vi "Read Boolean Channel Properties.vi"(7 "Input?":bool, 8 "error in (no error)":errorcluster, 10 "Bool Channel ID":string, 11 "Channel in":refnum<class "Channel.lvclass">) -> (0 "error out":errorcluster, 2 "Boolean Channel":T1, 3 "Channel out":refnum<class "Channel.lvclass">)   [LabVIEW 2026, in "Modbus.lvlib" / "Modbus.lvclass"]
uses:
  Modbus.lvclass
  <vilib>/FlexLogger/SDK/PluginSDK.lvlibp/PEFClasses/SDK/Channel/Channel.lvclass
  Types/Boolean Data.ctl
  Types/Modbus Table.ctl
  Globals/Modbus Strings.vi
  <vilib>/FlexLogger/SDK/PluginSDK.lvlibp/PEFClasses/SDK/Channel/ParameterAccess/Read Enum.vi
  <vilib>/FlexLogger/SDK/PluginSDK.lvlibp/PEFClasses/SDK/Channel/ParameterAccess/Read I32.vi
  <vilib>/FlexLogger/SDK/PluginSDK.lvlibp/PEFClasses/SDK/Channel/Read Valid.vi
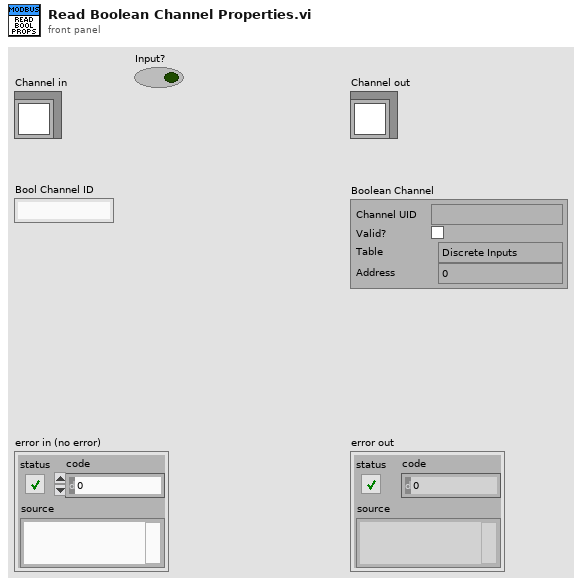
[diagram p1: front panel]
types:
  T1 = typedef "Modbus.lvlib/Modbus.lvclass/Boolean Data.ctl" = cluster{"Channel UID":string, "Valid?":bool, "Table":T2, "Address":i32}
  T2 = typedef "Modbus.lvlib/Modbus.lvclass/Modbus Table.ctl" = enum16{"Discrete Inputs", "Coils", "Input Registers", "Holding Registers"}
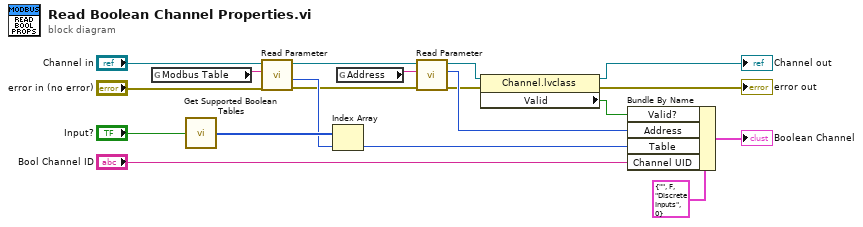
[diagram p0: block diagram]
diagram:
  n1 = global read "Modbus Strings.vi" "Modbus Table"() -> (w11:string)
  n2 = call "Get Supported Boolean Tables.vi"("Input?"="Input?") -> ("Supported Tables"=w19:T2[])
  n3 = call-poly <vilib>:"Read Parameter.vi"("error in (no error)"="error in (no error)", "Name"=w11, "Channel in"="Channel in") -> ("error out"=w13:errorcluster, "Index"=w15:i32, "Channel out"=w12:refnum<class "Channel.lvclass">)  [unwired: 4 in, 2 out]
  n4 = Index Array(array=w19, index=w15) -> (element=w16:T2)
  n5 = global read "Modbus Strings.vi" "Address"() -> (w14:string)
  n6 = call-poly <vilib>:"Read Parameter.vi"("error in (no error)"=w13, "Name"=w14, "Channel in"=w12) -> ("error out"=w6:errorcluster, "Value"=w17:i32, "Channel out"=w5:refnum<class "Channel.lvclass">)  [unwired: 5 in, 1 out]
  n7 = property class="Channel.lvclass"(reference=w5, error in=w6) -> (reference out=→"Channel out":refnum<class "Channel.lvclass">, error out=→"error out":errorcluster, "Valid"=w4:bool)
  n8 = Bundle By Name(cluster=T1 {"Channel UID"="", "Valid?"=FALSE, "Table"=enum."Discrete Inputs", "Address"=0} ("Boolean Data"), "Valid?"=w4, "Address"=w17, "Table"=w16, "Channel UID"="Bool Channel ID") -> (→"Boolean Channel":T1)
